vi "Write Batch Values - Variant.vi"(8 "error in (no error)":errorcluster, 10 "Array":variant[](array[variant]), 11 "OD Batch in":refnum<class "OD Batch.lvclass">) -> (0 "error out":errorcluster, 3 "OD Batch out":refnum<class "OD Batch.lvclass">)   [LabVIEW 2023, in "xnet_canopen.lvlib" / "OD Batch.lvclass"]
doc: "Expect OD Vars are all numeric types.\n\nFor I64 and U64, use <b>Type Cast</b> to restore exact value from double; For other types, use directly conversion."
uses:
  OD Batch.lvclass
  OD Batch.lvclass/OD Batch.ctl
  Write Batch OD By Array Index - bool.vi
  Write Batch OD By Array Index - i8.vi
  Write Batch OD By Array Index - i16.vi
  Write Batch OD By Array Index - i32.vi
  Write Batch OD By Array Index - u8.vi
  Write Batch OD By Array Index - u16.vi
  Write Batch OD By Array Index - u32.vi
  Write Batch OD By Array Index - f32.vi
  Write Batch OD By Array Index - string.vi
  Write Batch OD By Array Index - bytes.vi
  Write Batch OD By Array Index - f64.vi
  Write Batch OD By Array Index - i64.vi
  Write Batch OD By Array Index - u64.vi
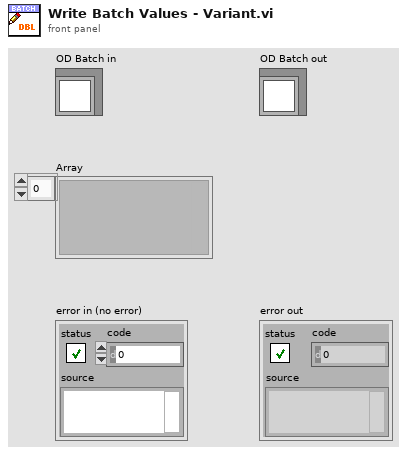
[diagram p1: front panel]
types:
  T1 = typedef "xnet_canopen.lvlib/od entry.ctl" = cluster{"OD Index":T2, "CANOpen Types":T3, "Size":u32, "Offset":u32, "Value":variant, "Initialized":bool}
  T2 = typedef "xnet_canopen.lvlib/od index.ctl" = cluster{"Index":u16, "SubIndex":u8}
  T3 = typedef "xnet_canopen.lvlib/canopen types.ctl" = u32
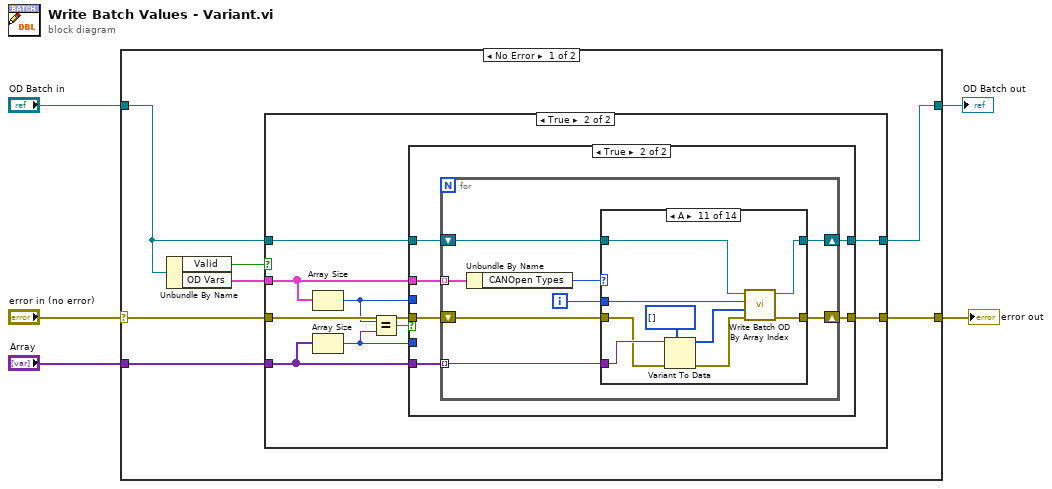
[diagram p0: block diagram]
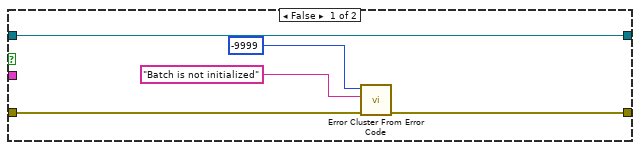
[diagram p2: hidden frame]
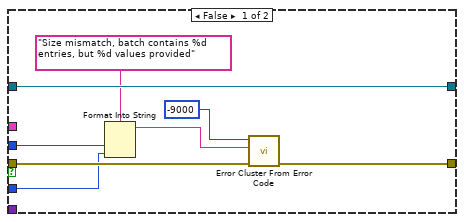
[diagram p3: hidden frame]
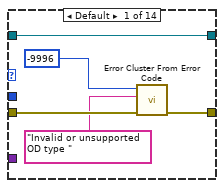
[diagram p4: hidden frame]
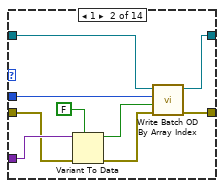
[diagram p5: hidden frame]
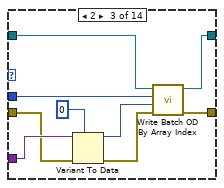
[diagram p6: hidden frame]
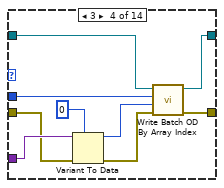
[diagram p7: hidden frame]
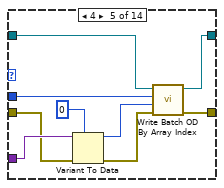
[diagram p8: hidden frame]
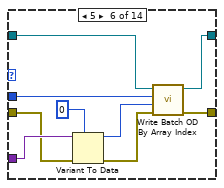
[diagram p9: hidden frame]
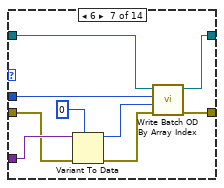
[diagram p10: hidden frame]
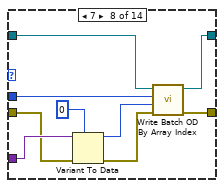
[diagram p11: hidden frame]
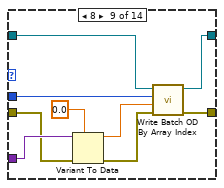
[diagram p12: hidden frame]
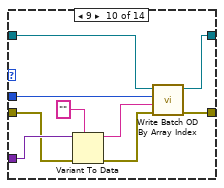
[diagram p13: hidden frame]
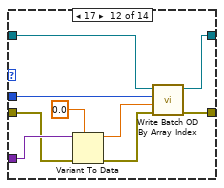
[diagram p14: hidden frame]
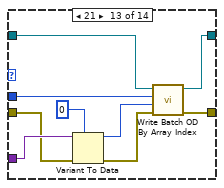
[diagram p15: hidden frame]
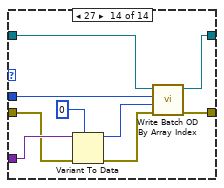
[diagram p16: hidden frame]
diagram:
  n1 = case shown="No Error" "error in (no error)" {
    selector: "error in (no error)" -> [w12 w171]
    tunnel: [w11 w171] -> w4
    tunnel: [w6 w172] -> w2
    tunnel: "OD Batch in" -> [w9 w172]
    tunnel: "Array" -> [w7 _]
    frame No Error {
      n2 = Unbundle By Name(w9) -> ("Valid"=w8:bool, "OD Vars"=w10:T1[])
      n3 = case shown="True" w8 {
        tunnel: w12 -> [w15 w26]
        tunnel: [w14 w25] -> w11
        tunnel: w10 -> [_ w22]
        tunnel: w9 -> [w13 w24]
        tunnel: w7 -> [_ w21]
        tunnel: [w13 w23] -> w6
        frame False {
          n4 = call <vilib>:"Error Cluster From Error Code.vi"("error in (no error)"=w15, "error message (\"\")"="Batch is not initialized" ("error message (\"\")"), "error code (0)"=-9999) -> ("error out"=w14:errorcluster)  [unwired: 6 in]
        }
        frame True {
          n5 = Array Size(array=w22) -> (size(s)=w18:i32)
          n6 = Array Size(array=w21) -> (size(s)=w19:i32)
          n7 = Equal?(x=w18, y=w19) -> (x = y?=w20:bool)
          n8 = case shown="True" w20 {
            tunnel: w26 -> [w34 w40]
            tunnel: [w32 w39] -> w25
            tunnel: w22 -> [_ w38]
            tunnel: w24 -> [w33 w37]
            tunnel: w21 -> [_ w36]
            tunnel: [w33 w35] -> w23
            tunnel: w19 -> [w29 _]
            tunnel: w18 -> [w28 _]
            frame False {
              n9 = Format Into String(format string="Size mismatch, batch contains %d entries, but %d values provided", w28, w29) -> (resulting string=w27:string)  [unwired: 2 in, 1 out]
              n10 = call <vilib>:"Error Cluster From Error Code.vi"("error in (no error)"=w34, "error message (\"\")"=w27, "error code (0)"=-9000) -> ("error out"=w32:errorcluster)  [unwired: 6 in]
            }
            frame True {
              n11 = for {
                shift-right: [w47] -> w39
                shift-left: w40 -> [w48]
                tunnel: w38 -> [w46] mode=indexing
                shift-right: [w41] -> w35
                shift-left: w37 -> [w43]
                tunnel: w36 -> [w42] mode=indexing
                i -> [w44]
                n12 = Unbundle By Name(w46) -> ("CANOpen Types"=w45:T3)
                n13 = case shown="A" w45 {
                  tunnel: w48 -> [w53 w57 w66 w75 w84 w93 w102 w111 w120 w129 w138 w147 w156 w165]
                  tunnel: [w52 w62 w71 w80 w89 w98 w107 w116 w125 w134 w143 w152 w161 w170] -> w47
                  tunnel: w44 -> [_ w61 w70 w79 w88 w97 w106 w115 w124 w133 w142 w151 w160 w169]
                  tunnel: w43 -> [w49 w60 w69 w78 w87 w96 w105 w114 w123 w132 w141 w150 w159 w168]
                  tunnel: w42 -> [_ w58 w67 w76 w85 w94 w103 w112 w121 w130 w139 w148 w157 w166]
                  tunnel: [w49 w59 w68 w77 w86 w95 w104 w113 w122 w131 w140 w149 w158 w167] -> w41
                  frame Default {
                    n14 = call <vilib>:"Error Cluster From Error Code.vi"("error in (no error)"=w53, "error message (\"\")"="Invalid or unsupported OD type " ("error message (\"\")"), "error code (0)"=-9996) -> ("error out"=w52:errorcluster)  [unwired: 6 in]
                  }
                  frame 1 {
                    n15 = Variant To Data(error in=w57, type=FALSE, Variant=w58) -> (data=w54:bool, error out=w56:errorcluster)
                    n16 = call-poly "Write Batch OD By Array Index.vi"("error in (no error)"=w56, "value"=w54, "array index"=w61, "OD Batch in"=w60) -> ("error out"=w62:errorcluster, "OD Batch out"=w59:refnum<class "OD Batch.lvclass">)  [unwired: 6 in]
                  }
                  frame 2 {
                    n17 = Variant To Data(error in=w66, type=i8 0, Variant=w67) -> (data=w63:i8, error out=w65:errorcluster)
                    n18 = call-poly "Write Batch OD By Array Index.vi"("error in (no error)"=w65, "value"=w63, "array index"=w70, "OD Batch in"=w69) -> ("error out"=w71:errorcluster, "OD Batch out"=w68:refnum<class "OD Batch.lvclass">)  [unwired: 6 in]
                  }
                  frame 3 {
                    n19 = Variant To Data(error in=w75, type=i16 0, Variant=w76) -> (data=w72:i16, error out=w74:errorcluster)
                    n20 = call-poly "Write Batch OD By Array Index.vi"("error in (no error)"=w74, "value"=w72, "array index"=w79, "OD Batch in"=w78) -> ("error out"=w80:errorcluster, "OD Batch out"=w77:refnum<class "OD Batch.lvclass">)  [unwired: 6 in]
                  }
                  frame 4 {
                    n21 = Variant To Data(error in=w84, type=0, Variant=w85) -> (data=w81:i32, error out=w83:errorcluster)
                    n22 = call-poly "Write Batch OD By Array Index.vi"("error in (no error)"=w83, "value"=w81, "array index"=w88, "OD Batch in"=w87) -> ("error out"=w89:errorcluster, "OD Batch out"=w86:refnum<class "OD Batch.lvclass">)  [unwired: 6 in]
                  }
                  frame 5 {
                    n23 = Variant To Data(error in=w93, type=u8 0, Variant=w94) -> (data=w90:u8, error out=w92:errorcluster)
                    n24 = call-poly "Write Batch OD By Array Index.vi"("error in (no error)"=w92, "value"=w90, "array index"=w97, "OD Batch in"=w96) -> ("error out"=w98:errorcluster, "OD Batch out"=w95:refnum<class "OD Batch.lvclass">)  [unwired: 6 in]
                  }
                  frame 6 {
                    n25 = Variant To Data(error in=w102, type=u16 0, Variant=w103) -> (data=w99:u16, error out=w101:errorcluster)
                    n26 = call-poly "Write Batch OD By Array Index.vi"("error in (no error)"=w101, "value"=w99, "array index"=w106, "OD Batch in"=w105) -> ("error out"=w107:errorcluster, "OD Batch out"=w104:refnum<class "OD Batch.lvclass">)  [unwired: 6 in]
                  }
                  frame 7 {
                    n27 = Variant To Data(error in=w111, type=u32 0, Variant=w112) -> (data=w108:u32, error out=w110:errorcluster)
                    n28 = call-poly "Write Batch OD By Array Index.vi"("error in (no error)"=w110, "value"=w108, "array index"=w115, "OD Batch in"=w114) -> ("error out"=w116:errorcluster, "OD Batch out"=w113:refnum<class "OD Batch.lvclass">)  [unwired: 6 in]
                  }
                  frame 8 {
                    n29 = Variant To Data(error in=w120, type=sgl 0.0, Variant=w121) -> (data=w117:sgl, error out=w119:errorcluster)
                    n30 = call-poly "Write Batch OD By Array Index.vi"("error in (no error)"=w119, "value"=w117, "array index"=w124, "OD Batch in"=w123) -> ("error out"=w125:errorcluster, "OD Batch out"=w122:refnum<class "OD Batch.lvclass">)  [unwired: 6 in]
                  }
                  frame 9 {
                    n31 = Variant To Data(error in=w129, type="", Variant=w130) -> (data=w126:string, error out=w128:errorcluster)
                    n32 = call-poly "Write Batch OD By Array Index.vi"("error in (no error)"=w128, "value"=w126, "array index"=w133, "OD Batch in"=w132) -> ("error out"=w134:errorcluster, "OD Batch out"=w131:refnum<class "OD Batch.lvclass">)  [unwired: 6 in]
                  }
                  frame 10 {
                    n33 = Variant To Data(error in=w138, type=u8[] [], Variant=w139) -> (data=w135:u8[], error out=w137:errorcluster)
                    n34 = call-poly "Write Batch OD By Array Index.vi"("error in (no error)"=w137, "value"=w135, "array index"=w142, "OD Batch in"=w141) -> ("error out"=w143:errorcluster, "OD Batch out"=w140:refnum<class "OD Batch.lvclass">)  [unwired: 6 in]
                  }
                  frame 17 {
                    n35 = Variant To Data(error in=w147, type=0.0, Variant=w148) -> (data=w144:dbl, error out=w146:errorcluster)
                    n36 = call-poly "Write Batch OD By Array Index.vi"("error in (no error)"=w146, "value"=w144, "array index"=w151, "OD Batch in"=w150) -> ("error out"=w152:errorcluster, "OD Batch out"=w149:refnum<class "OD Batch.lvclass">)  [unwired: 6 in]
                  }
                  frame 21 {
                    n37 = Variant To Data(error in=w156, type=i64 0, Variant=w157) -> (data=w153:i64, error out=w155:errorcluster)
                    n38 = call-poly "Write Batch OD By Array Index.vi"("error in (no error)"=w155, "value"=w153, "array index"=w160, "OD Batch in"=w159) -> ("error out"=w161:errorcluster, "OD Batch out"=w158:refnum<class "OD Batch.lvclass">)  [unwired: 6 in]
                  }
                  frame 27 {
                    n39 = Variant To Data(error in=w165, type=u64 0, Variant=w166) -> (data=w162:u64, error out=w164:errorcluster)
                    n40 = call-poly "Write Batch OD By Array Index.vi"("error in (no error)"=w164, "value"=w162, "array index"=w169, "OD Batch in"=w168) -> ("error out"=w170:errorcluster, "OD Batch out"=w167:refnum<class "OD Batch.lvclass">)  [unwired: 6 in]
                  }
                }
              }
            }
          }
        }
      }
    }
    frame Error {
    }
  }
  "error out" <- w4
  "OD Batch out" <- w2
